vi "Write TAI Start Time (ns).vi"(8 "error in (no error)":errorcluster, 10 "TAI Start Time (ns)":i64, 11 "XNET CAN RW in":refnum<class "XNET CAN RW.lvclass">) -> (0 "error out":errorcluster, 3 "XNET CAN RW out":refnum<class "XNET CAN RW.lvclass">)   [LabVIEW 2021, in "XNET CAN RW.lvclass"]
uses:
  XNET CAN RW.lvclass
  XNET CAN RW.lvclass/XNET CAN RW.ctl
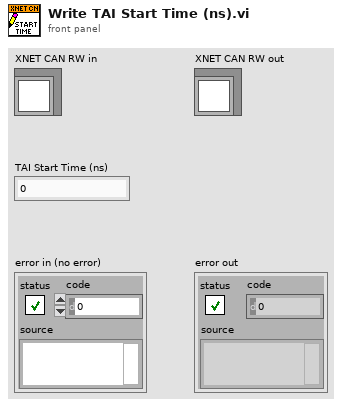
[diagram p1: front panel]
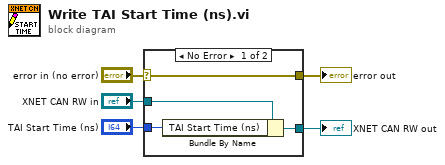
[diagram p0: block diagram]
diagram:
  n1 = case shown="No Error" "error in (no error)" {
    selector: "error in (no error)" -> [w9 w10]
    tunnel: [w9 w10] -> w4
    tunnel: [w7 w11] -> w2
    tunnel: "XNET CAN RW in" -> [w8 w11]
    tunnel: "TAI Start Time (ns)" -> [w6 _]
    frame No Error {
      n2 = Bundle By Name(cluster=w8, "TAI Start Time (ns)"=w6) -> (w7:refnum<class "XNET CAN RW.lvclass">)
    }
    frame Error {
    }
  }
  "error out" <- w4
  "XNET CAN RW out" <- w2
